vi "SUP_Camera_SetupObserve.vi"(5 "error in (no error)":errorcluster, 6 "Image":T1, 7 "valeur de l'horloge en ms 3":u32, 8 "SetupOK":bool, 9 "valeur de l'horloge en ms 2":u32, 10 "temps actuel":timestamp, 11 "valeur de l'horloge en ms":u32) -> (0 "valid_for_run":bool, 1 "channel_out":u32, 2 "capture":timestamp, 3 "error in (no error) 2":errorcluster, 4 "Image 2":T1)   [LabVIEW 2012]
uses:
  <vilib>/vision/Image Controls.llb/IMAQ Image.ctl
panel:
  in  "temps actuel 3":timestamp
  out "error in (no error) 3":errorcluster
  in  "temps actuel 2":timestamp
  out "Image Pixels (I16)":i16[][](array[numeric])
  out "Image Pixels (U8)":u8[][](array[numeric])
  out "error out":errorcluster
  out "Image Pixels (Float)":sgl[][](array[numeric]) format="%.2f"
  out "Image Pixels (U16)":u16[][](array[numeric])
  in  "Optional Rectangle":i32[](array[numeric])
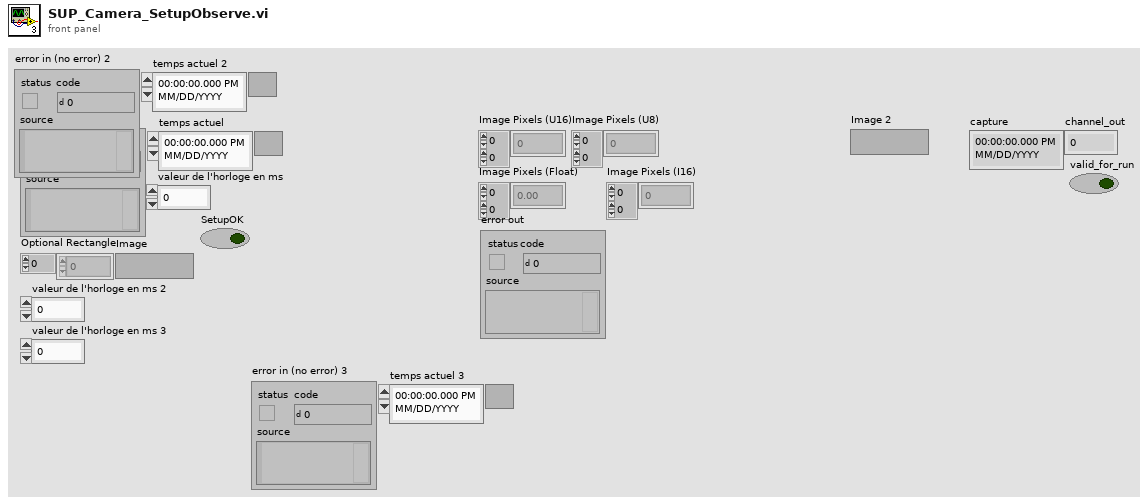
[diagram p1: front panel]
types:
  T1 = typedef "IMAQ Image.ctl" = refnum<image>
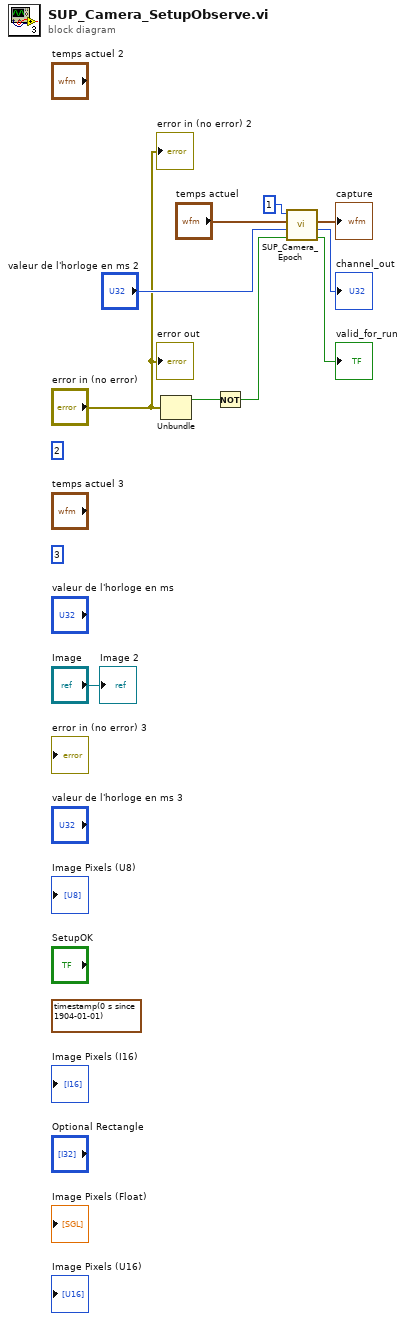
[diagram p0: block diagram]
diagram:
  (unwired) u32 3 ("valeur de l'horloge en ms 2")
  (unwired) u32 2 ("valeur de l'horloge en ms 2")
  (unwired) timestamp(0 s since 1904-01-01) ("temps actuel 3")
  n1 = Unbundle("error in (no error)") -> ("status"=w5:bool)  [unwired: 2 out]
  n2 = Not(x=w5) -> (.not. x?=w4:bool)
  n3 = call "SUP_Camera_Epoch.vi"("SetupOK"=w4, "valeur de l'horloge en ms 2"="valeur de l'horloge en ms 2", "temps actuel"="temps actuel", "valeur de l'horloge en ms"=u32 1 ("valeur de l'horloge en ms 2")) -> ("valid_for_run"=→"valid_for_run":bool, "channel_out"=→"channel_out":u32, "capture"=→"capture":timestamp)  [unwired: 3 in, 2 out]
  "error out" <- "error in (no error)"
  "error in (no error) 2" <- "error in (no error)"
  "Image 2" <- "Image"
